vi "LoadKeyboardLUT.vi"(11 "Metadata":T1[](array[typedef])) -> (0 "error out":errorcluster, 3 "Samples":u32)   [LabVIEW 2026, in "dependencies.lvlib"]
uses:
  dependencies.lvlib
  KeyboardLUTSelector.ctl
  KeyboardAndMouseDataAcquisition.ctl
  KeyType.ctl
panel:
  # "wqeeeeeeeeeeeeeeeeeeeeeeeeeeeeeeeeeeeeeeeeeeeeeeeeeeeeeeeeeeeeeeeeeeeeeeeeeeeeee"
  # "sssssssssssssddddddddddddddddddddddddddddddddddddddddddd"
  # "fsdsdsdsdsdsdsdsdsdsdaaaaaaaaaaaaaaaaaaaaaaaaaaaaaaaaa"
  # "qweeeeeeeeewqqqqqqqqqqqqqqqqqqqqqqqqqqqqqqqqqqqqqqqqqq"
  # "sdffffffffffffffffffAAAAAA"
  # "sdsdsdsdsdsdsdsdsdsdaaaaaaaaaaaaaaaaaaaaaaaaaaaaaaaaaaaaaaaaaaaaaaaaaaaaaaaaaaa"
  # "rewwwwwwwwwwwwwwwwwwwwrewwerrrrrrrrrewwwwwwwwwwwwww"
  # "rew"
  # "rrrrrrrrreeeeeeeewwwwwwwwww"
  # "rrrrrrrreeeeeeeeeeewwwwwwwwwwwwwww"
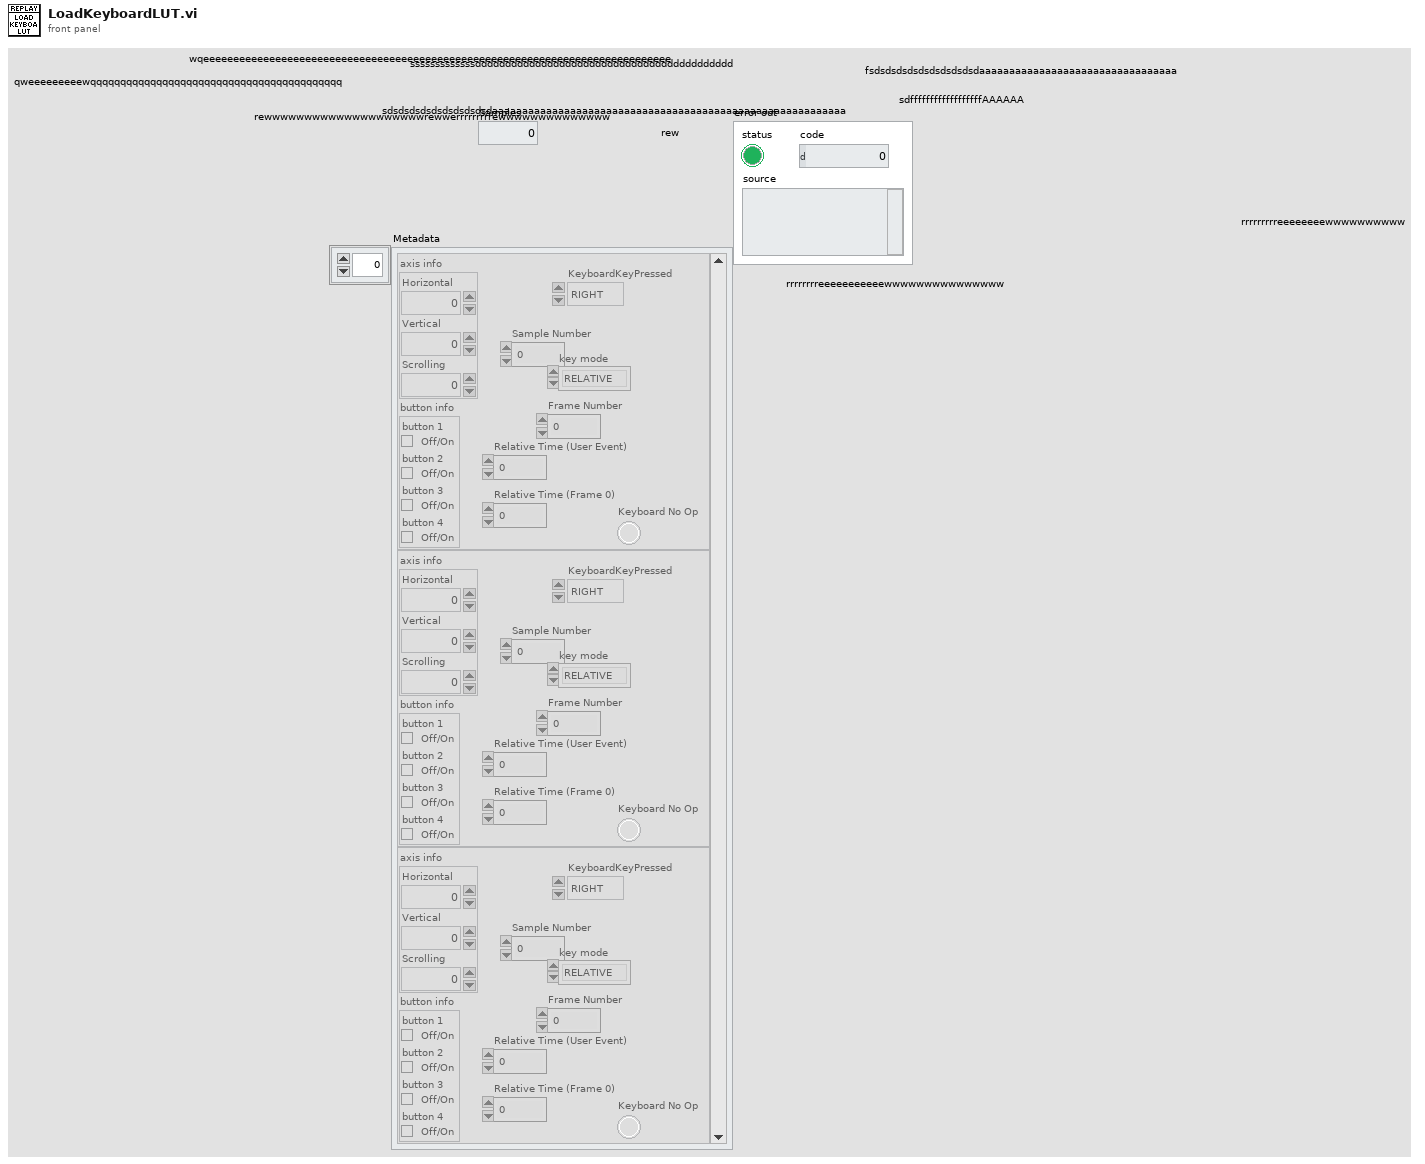
[diagram p1: front panel]
types:
  T1 = typedef "dependencies.lvlib/KeyboardAndMouseDataAcquisition.ctl" = cluster{"axis info":cluster{"Horizontal":i32, "Vertical":i32, "Scrolling":i32}, "button info":cluster{"button 1":bool, "button 2":bool, "button 3":bool, "button 4":bool}, "Relative Time (User Event)":dbl, "Sample Number":u32, "Relative Time (Frame 0)":dbl, "key mode":enum16{"RELATIVE", "ABSOLUTE"}, "Frame Number":u32, "KeyboardKeyPressed":T2, "Keyboard No Op":bool}
  T2 = typedef "dependencies.lvlib/KeyType.ctl" = enum16{"0", "1", "2", "3", "4", "5", "6", "7", "8", "9", "A", "B", "C", "D", "E", "F", "G", "H", "I", "J", "K", "L", "M", "N", "O", "P", "Q", "R", "S", "T", "U", "V", "W", "X", "Y", "Z", "F1", "F2", "F3", "F4", "F5", "F6", "F7", "F8", "F9", "F10", "F11", "F12", "F13", "F14", "F15", "ADD", "BACK", "BACKSLASH", "CAPITAL", "COMMA", "DECIMAL", "DELETE", "DIVIDE", "DOWN", "END", "EQUALS", "ESCAPE", "GRAVE (`)", "HOME", "INSERT", "LBRACKET", "LCONTROL", "LEFT", "L ALT", "LSHIFT", "LWIN", "MINUS", "MULTIPLY", "NEXT", "NUMLOCK", "NUMPAD_0", "NUMPAD_1", "NUMPAD_2", "NUMPAD_3", "NUMPAD_4", "NUMPAD_5", "NUMPAD_6", "NUMPAD_7", "NUMPAD_8", "NUMPAD_9", "PAUSE", "PERIOD", "PRIOR (PG UP)", "RBRACKET", "RCONTROL", "RETURN", "RIGHT", "R ALT", "RSHIFT", "RWIN", "SCROLL", "SEMICOLON", "SLASH", "SPACE", "SUBTRACT", "TAB", "UP", "ENTER (num pad)", "' (quote)"}
  T3 = typedef "dependencies.lvlib/KeyboardLUTSelector.ctl" = enum16{"Initialize", "Get Keyboards Keys Pressed at Sample Number", "Assign Keyboard Key Press to Sample Number"}
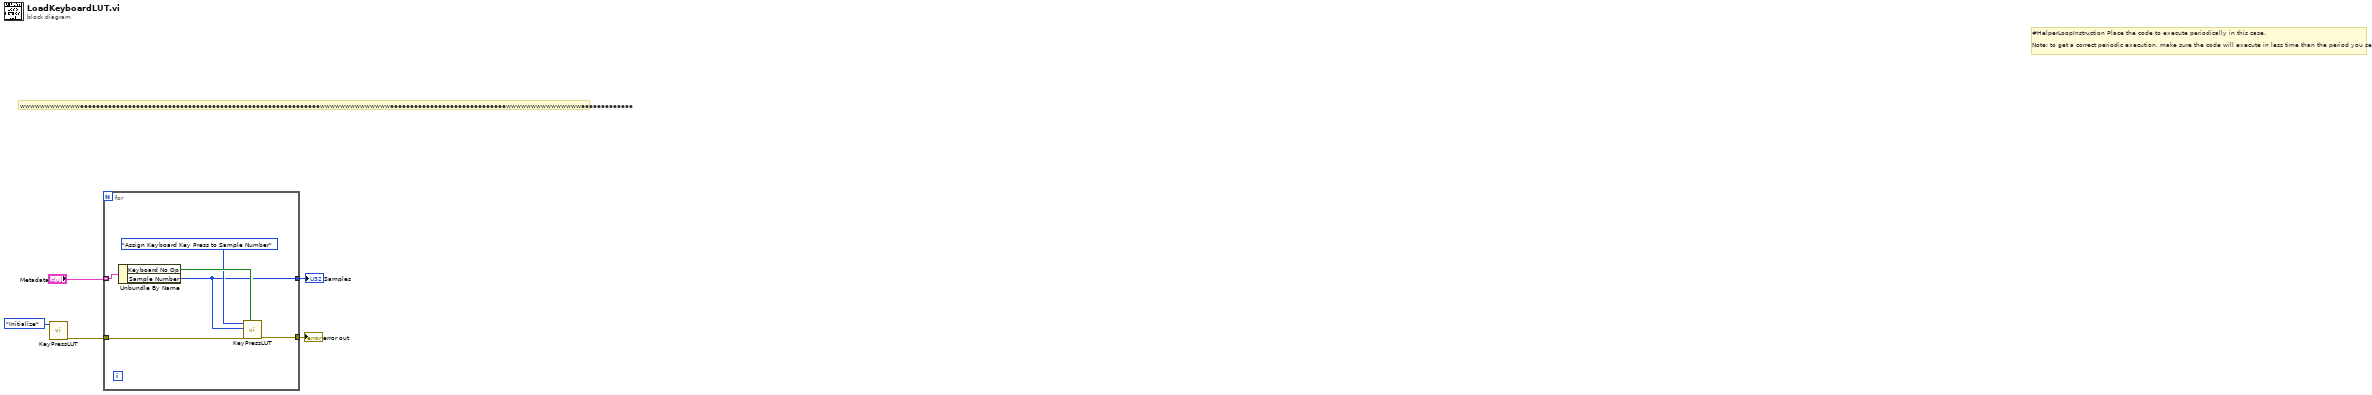
[diagram p0: block diagram]
diagram:
  # "#HelperLoopInstruction Place the code to execute periodically in this case.\n\nNote: to get a correct periodic execution, make sure the code will execute in less time than the period you set."
  # "wwwwwwwwwwwweeeeeeeeeeeeeeeeeeeeeeeeeeeeeeeeeeeeeeeeeeeeeeeeeeeeeeeeeeeewwwwwwwwwwwwwweeeeeeeeeeeeeeeeeeeeeeeeeeeeewwwwwwwwwwwwwwweeeeeeeeeeeee"
  n1 = call "KeyPressLUT.vi"("LUT Selector"=KeyboardLUTSelector."Initialize") -> ("error out"=w4:errorcluster)  [unwired: 9 in, 1 out]
  n2 = for {
    tunnel: "Metadata" -> [w11] mode=indexing
    tunnel: w4 -> [w8]
    tunnel: [w7] -> w2
    tunnel: [w6] -> w1
    n3 = Unbundle By Name(w11) -> ("Keyboard No Op"=w10:bool, "Sample Number"=w6:u32)
    n4 = call "KeyPressLUT.vi"("Keyboard No Op"=w10, "error in (no error)"=w8, "Sample Number"=w6, "LUT Selector"=KeyboardLUTSelector."Assign Keyboard Key Press to Sample Number") -> ("error out"=w7:errorcluster)  [unwired: 6 in, 1 out]
  }
  "error out" <- w2
  "Samples" <- w1
